vi "RemoteVI Close Window.vi"(0 "kind":T2(ring), 5 "id":u64, 7 "windows":T1(array[cluster]), 11 "error in":errorcluster) -> (4 "closed?":bool, 15 "error out":errorcluster)   [LabVIEW 2020, in "RemoteVI.lvlib"]
doc: "Handles the client message x <id> (docs\\protocol.md section 7): when kind is close and id is a LISTED window whose closable flag is set (it has a close box, WS_SYSMENU), WM_SYSCOMMAND (0x112) with SC_CLOSE (0xF060) is posted to it with user32 PostMessageW.vi - exactly what its title bar's close button sends, so the window closes the way it would locally (a native dialog cancels). A bare WM_CLOSE is NOT posted: measured on LabVIEW 2025, WM_CLOSE posted to a Two Button Dialog destroyed its window while the dialog function kept waiting for an answer, which hung the calling VI and LabVIEW's VI Server. Anything else does nothing: nothing goes to the published panel (it is not in windows) or to a window the server does not list, and no other message can be sent this way. closed? is TRUE when it was posted."
uses:
  RemoteVI.lvlib
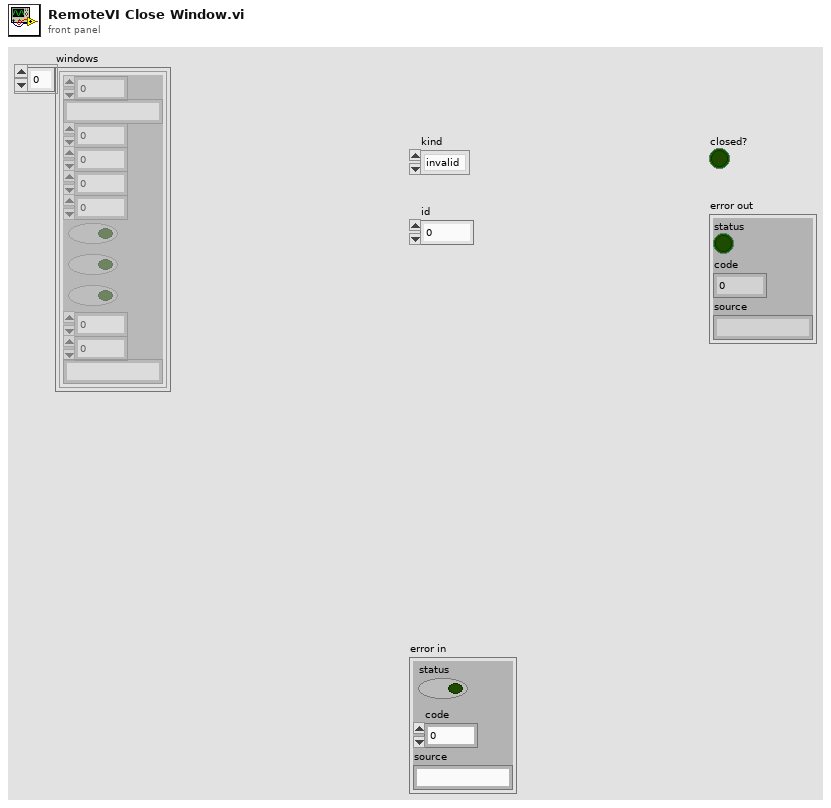
[diagram p1: front panel]
types:
  T1 = cluster{"id":u64, "title":string, "x":i32, "y":i32, "w":i32, "h":i32, "modal":bool, "active":bool, "closable":bool, "sx":i32, "sy":i32, "class":string}[]
  T2 = enum16{"invalid", "mouse", "key", "ack", "close", "splitter"}
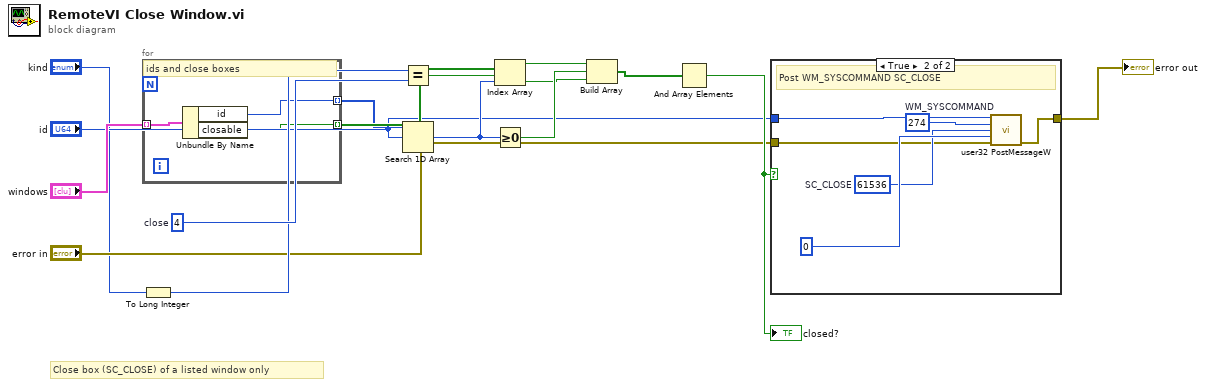
[diagram p0: block diagram]
diagram:
  w11 = 4  # close
  # "Close box (SC_CLOSE) of a listed window only"
  n1 = for {
    tunnel: "windows" -> [w16] mode=indexing
    tunnel: [w17] -> w5 mode=indexing
    tunnel: [w18] -> w6 mode=indexing
    # "ids and close boxes"
    n2 = Unbundle By Name(w16) -> ("id"=w17:u64, "closable"=w18:bool)
  }
  n3 = To Long Integer(number="kind") -> (32bit integer=w10:i32)
  n4 = Equal?(x=w10, y=w11) -> (x = y?=w12:bool)
  n5 = Search 1D Array(1D array=w5, element="id") -> (index of element=w7:i32)  [unwired: 1 in]
  n6 = Index Array(array=w6, index=w7) -> (element=w8:bool)
  n7 = Greater Or Equal To 0?(x=w7) -> (x >= 0?=w9:bool)
  n8 = Build Array(w12, w9, w8) -> (w13:bool[])
  n9 = And Array Elements(Boolean array=w13) -> (logical AND=w14:bool)
  "closed?" <- w14
  n10 = case shown="True" w14 {
    tunnel: "id" -> [_ w20]
    tunnel: "error in" -> [w19 w21]
    tunnel: [w19 w25] -> w15
    frame False {
      # "Not a listed, closable window"
    }
    frame True {
      w23 = u64 61536  # SC_CLOSE
      w22 = u32 274  # WM_SYSCOMMAND
      # "Post WM_SYSCOMMAND SC_CLOSE"
      n11 = call "user32 PostMessageW.vi"("hWnd"=w20, "Msg"=w22, "wParam"=w23, "lParam"=i64 0, "error in (no error)"=w21) -> ("error out"=w25:errorcluster)  [unwired: 9 in, 1 out]
    }
  }
  "error out" <- w15
